vi "test0509.vi"() -> ()   [LabVIEW 2019]
panel:
  out "error out":errorcluster
  in  "error in (no error)":errorcluster
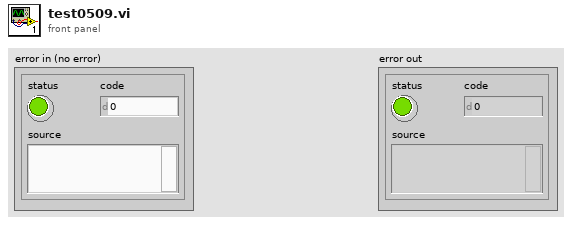
[diagram p1: front panel]
types:
  T1 = enum16{"向前校正", "向後校正", "右後校正", "右前校正", "左前校正", "左後校正", ""}
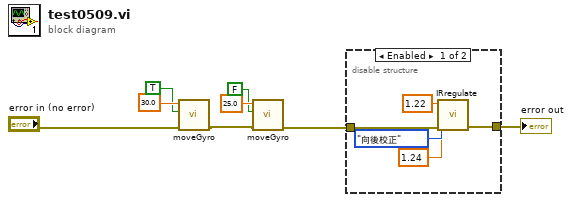
[diagram p0: block diagram]
diagram:
  n1 = call "moveGyro.vi"("error in (no error)"="error in (no error)", "タは"=TRUE, "移動距離"=30.0) -> ("error out"=w5:errorcluster)  [unwired: 8 in]
  n2 = call "moveGyro.vi"("error in (no error)"=w5, "タは"=FALSE, "移動距離"=25.0) -> ("error out"=w4:errorcluster)  [unwired: 8 in]
  n3 = disable-structure shown="Enabled" {
    disable-tunnel: [w13 _] -> w8
    disable-tunnel: w4 -> [w9 _]
    frame Enabled {
      n4 = call "IRregulate.vi"("error in (no error)"=w9, "Enum"=T1."向後校正", "左後距離"=1.24, "右後距離"=1.22) -> ("error out"=w13:errorcluster)  [unwired: 7 in]
    }
    frame Disabled {
    }
  }
  "error out" <- w8
